vi "fake tool name clash.vi"(10 "a_b":i32, 11 "a b":i32) -> (3 "sum":i32)   [LabVIEW 2020, in "MCP Server tests.lvlib"]
doc: "This is a fake tool to test the MCP server toolkit. Its two inputs are labelled a b and a_b, which both map to the MCP name a_b, so Add Tool.vi must refuse to register it."
uses:
  MCP Server tests.lvlib
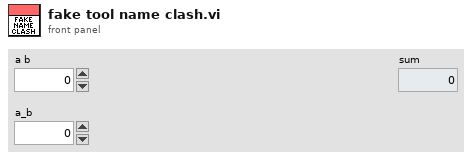
[diagram p1: front panel]
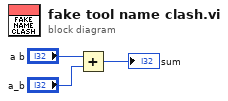
[diagram p0: block diagram]
diagram:
  n1 = Add(x="a b", y="a_b") -> (x+y=→"sum":i32)
